vi "VM - DBL Scalar.vi"(6 "global? (F)":bool, 7 "VC Handle":T3=-1, 8 "error in":errorcluster, 9 "cmd":T2(ring)=enum."get value", 10 "value in":dbl, 11 "name_spec":string) -> (0 "error out":errorcluster, 1 "err code":T1 items=["No error", "Invalid variable type", "Variable not found", "Variable already exists", "Invalid context handle", "Input error", "Invalid data format", "No history attached", "History already attached", "Invalid history parameters", "Wrong variable name", "Wrong alias name", "Non-unique alias", "Alias not found", "No alias associated", "Alias already associated", "Wrong context name", "Non-unique context name", "Context name not found", "Invalid parameter", "Generic error", "Memory Full", "Unrecognized LV error", "Unknown error code"], 2 "value out":dbl, 3 "dup name_spec":string, 4 "global out":bool, 5 "dup VC Handle":T3=-1)   [LabVIEW 2021]
doc: "This VI manages variables of the <b>DBL Number</b> data type. Refer to the VI help for more details.\n\n<b>VC Handle</b> specifies the handle of the variable context. This input is ignored if the <b>name_spec</b> control refers to a variable by an alias during 'get value', 'set value', and 'destroy' actions or if the action is 'create' and <b>global?</b> is TRUE.\n\n<b>name_spec</b> is the name specifier of the desired variable. Usually, it is merely a variable name; however, its generic format is '[name][=alias]', where either 'name' or '=alias' can be omitted but not both.\n\n<b>cmd</b> control specifies the action to be performed on the variable. Possible actions are 'create', 'destroy', 'get value', and 'set value'.\n\n<b>value in</b> control specifies the value to be written to the variable; it is only used during 'set value' or 'create' actions. <b>value out</b> indicator returns the value that has been read from the variable.\n\n<b>global?</b> control, if TRUE, enables access to global variables. For 'create' and 'destroy' actions, it causes the VI to ignore <b>VC Handle</b> and operate on a global variable. For 'get value' and 'set value' actions, it allows the VI to operate on a global variable if the specified variable name is not found in the context specified by <b>VC Handle</b>.\n\n<b>global out</b> indicator returns TRUE if an action has been performed on a global variable.\n\n<b>err code</b> indicator returns a VarMan Engine error code.\n\n::: CalcExpress Toolkit :::\nCopyright (c) 2000-2026 Konstantin Shifershteyn. All rights reserved."
uses:
  cetypes.llb/VarMan Variable Context Handle.ctl
  cetypes.llb/VarMan Error Code.ctl
  cersrc/celveng32.dll
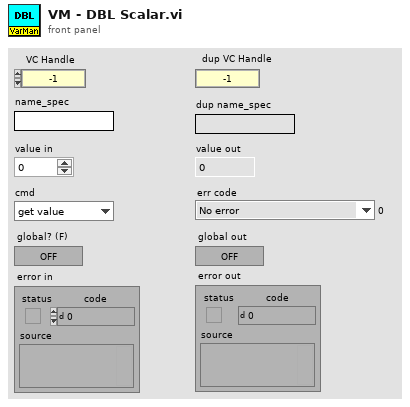
[diagram p1: front panel]
types:
  T1 = typedef "VarMan Error Code.ctl" = u16
  T2 = enum16{"create", "destroy", "set value", "get value"}
  T3 = typedef "VarMan Variable Context Handle.ctl" = i32
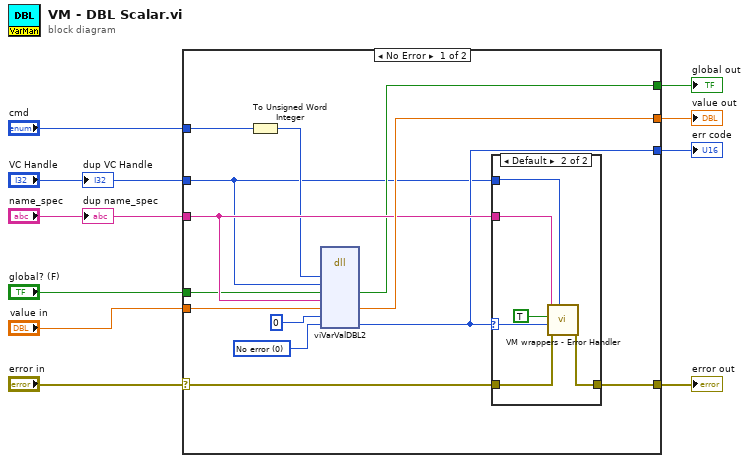
[diagram p0: block diagram]
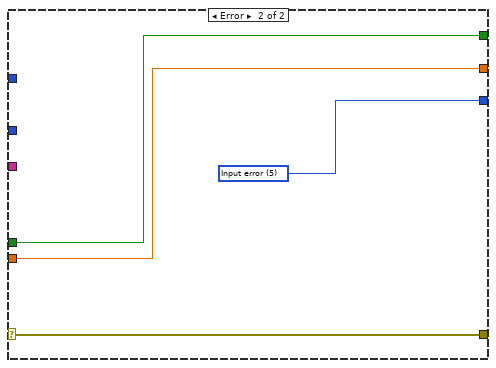
[diagram p3: hidden frame]
diagram:
  n1 = case shown="No Error" "error in" {
    selector: "error in" -> [w18 w34]
    tunnel: [w23 w32] -> w3
    tunnel: [w14 w31] -> w4
    tunnel: "value in" -> [w22 w32]
    tunnel: "cmd" -> [w21 _]
    tunnel: "name_spec" -> [w20 _]
    tunnel: "VC Handle" -> [w12 _]
    tunnel: [w19 w34] -> w5
    tunnel: "global? (F)" -> [w16 w33]
    tunnel: [w15 w33] -> w2
    frame No Error {
      w13 = T1 0 items=["No error", "Invalid variable type", "Variable not found", "Variable already exists", "Invalid context handle", "Input error", "Invalid data format", "No history attached", "History already attached", "Invalid history parameters", "Wrong variable name", "Wrong alias name", "Non-unique alias", "Alias not found", "No alias associated", "Alias already associated", "Wrong context name", "Non-unique context name", "Context name not found", "Invalid parameter", "Generic error", "Memory Full", "Unrecognized LV error", "Unknown error code"] ("err code")
      n2 = To Unsigned Word Integer(number=w21) -> (unsigned 16bit integer=w17:u16)
      n3 = dll-call lib="C:/LV Projects/CalcExpress 40 LV2021/vi.lib/addons/CalcExpress/cersrc/celveng*.dll" fn="viVarValDBL2"("cmd"=w17, "vch"=w12, "glob"=w16, "name"=w20, "value"=w22, "writerID"=u32 0, "errc"=w13) -> ("glob"=w15:bool, "value"=w23:dbl, "errc"=w14:T1)  [unwired: 8 in, 2 out]
      n4 = case shown="Default" w14 {
        selector: w14 -> [_ w25]
        tunnel: [w24 w30] -> w19
        tunnel: w18 -> [w24 w29]
        tunnel: w12 -> [_ w28]
        tunnel: w20 -> [_ w27]
        frame 0 {
        }
        frame Default {
          n5 = call "VM wrappers - Error Handler.vi"("VC Handle"=w28, "error before"=w29, "VarMan error"=w25, "show name spec (F)"=TRUE, "name spec"=w27) -> ("error out"=w30:errorcluster)  [unwired: 5 in, 1 out]
        }
      }
    }
    frame Error {
      w31 = T1 5 items=["No error", "Invalid variable type", "Variable not found", "Variable already exists", "Invalid context handle", "Input error", "Invalid data format", "No history attached", "History already attached", "Invalid history parameters", "Wrong variable name", "Wrong alias name", "Non-unique alias", "Alias not found", "No alias associated", "Alias already associated", "Wrong context name", "Non-unique context name", "Context name not found", "Invalid parameter", "Generic error", "Memory Full", "Unrecognized LV error", "Unknown error code"] ("err code")
    }
  }
  "value out" <- w3
  "error out" <- w5
  "err code" <- w4
  "global out" <- w2
  "dup VC Handle" <- "VC Handle"
  "dup name_spec" <- "name_spec"
